vi "UDP test Half 2.vi"() -> ()   [LabVIEW 2013, in "TEC tests.lvlib"]
uses:
  TEC tests.lvlib
  configuration/TEC configuration.lvclass
  execution/TEC runtime.lvclass
  <vilib>/NI/Module Timing Source/usec timing source/usec timing source.lvclass
  configuration/TEC configuration.lvclass/TEC configuration.ctl
  <vilib>/NI/Tag Bus/table/data polymorphs/read one/read Double.vi
  <vilib>/NI/Tag Bus/table/data polymorphs/read one/read Array of U64.vi
  configuration/Write receive on port.vi
  configuration/Write send from port.vi
  configuration/Write send to address.vi
  configuration/Write send to port.vi
  <vilib>/NI/Tag Bus/table/data table.lvlib
  <vilib>/ptbypt/NI_PtbyPt.lvlib
  <vilib>/NI/Configuration Framework/serializable configuration/NISE_CEF_serializable configuration.lvclass
panel:
  out "value":u64[](array[numeric])
  out "error out 2":errorcluster
  out "error out":errorcluster
  in  "send to address":string="dsmith"
  out "duration avg":dbl
  in  "dt":u32=100
  out "duration":dbl
  out "timeout count":u16
  out "final":errorcluster
  out "value rx":dbl
  in  "stop":bool
  out "init err":errorcluster
  in  "ch count":i32=100
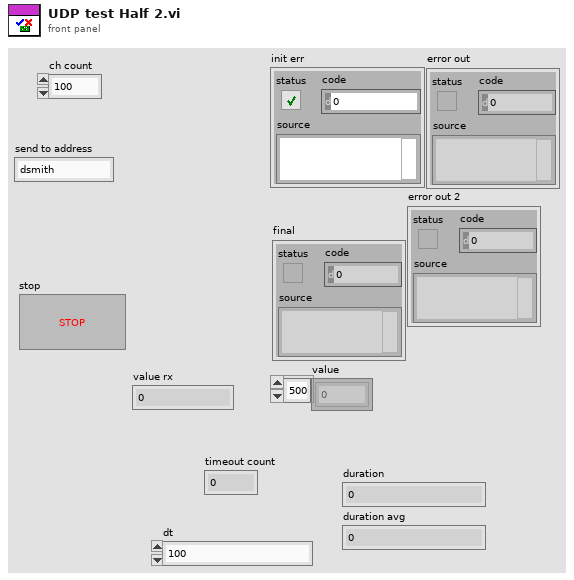
[diagram p1: front panel]
types:
  T1 = typedef "TBM channel.lvclass/data tables.ctl" = cluster{"input data":T2, "processing parameter":T2, "processing result":T2, "output data":T2}
  T2 = typedef "tag bus.lvlib/dictionary table pair.ctl" = cluster{"data dictionary":refnum<class "data dictionary.lvclass">, "data table":T3}
  T3 = typedef "tag bus.lvlib/data table.lvlib/data table.ctl" = cluster{"Double":dbl[], "Single":sgl[], "I64":i64[], "I32":i32[], "I16":i16[], "I8":i8[], "U64":u64[], "U32":u32[], "U16":u16[], "U8":u8[], "Boolean":bool[], "String":string[], "Array of Double":cluster{"DBL Array":dbl[]}[], "Array of Single":cluster{"SGL Array":sgl[]}[], "Array of I64":cluster{"I64 Array":i64[]}[], "Array of I32":cluster{"I32 Array":i32[]}[], "Array of I16":cluster{"I16 Array":i16[]}[], "Array of I8":cluster{"I8 Array":i8[]}[], "Array of U64":cluster{"U64 Array":u64[]}[], "Array of U32":cluster{"U32 Array":u32[]}[], "Array of U16":cluster{"U16 Array":u16[]}[], "Array of U8":cluster{"U8 Array":u8[]}[], "Array of Boolean":cluster{"Boolean Array":bool[]}[], "Array of String":cluster{"String Array":string[]}[]}
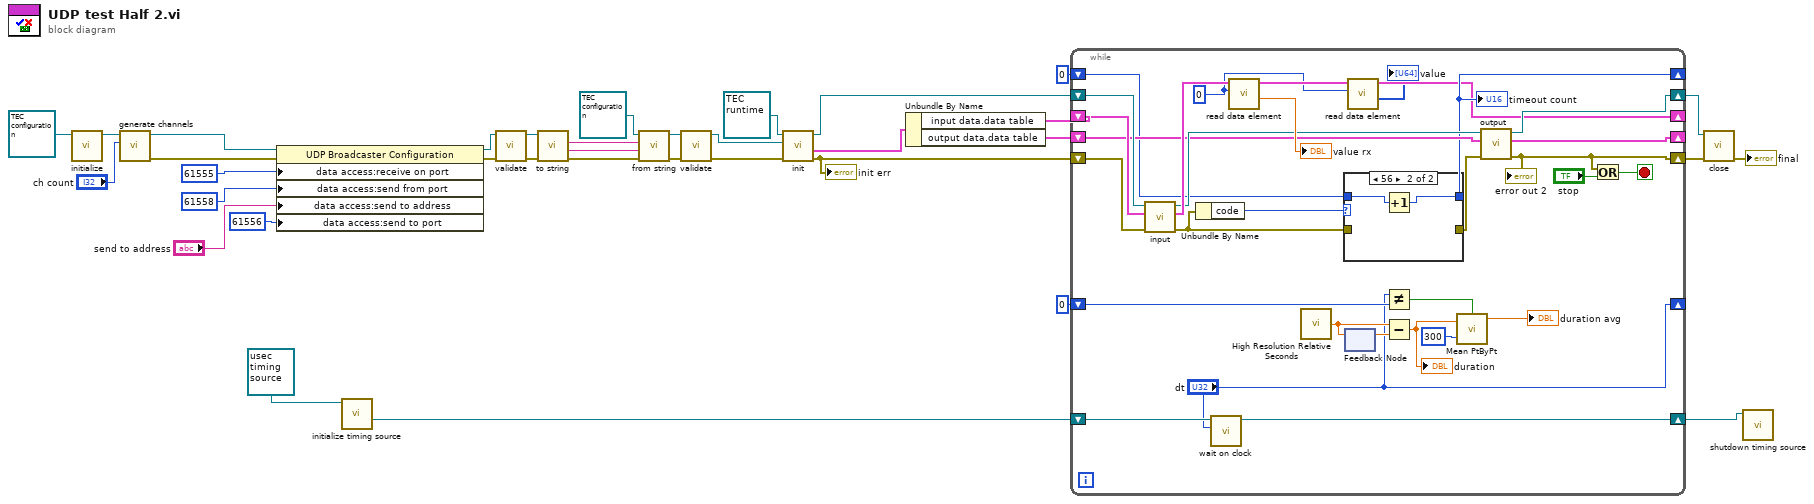
[diagram p0: block diagram]
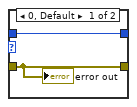
[diagram p2: hidden frame]
diagram:
  n1 = call <vilib>:"initialize.vi"("configuration in"=refnum<class "TEC configuration.lvclass"> refnum ("tag bus configurable plugin module configuration")) -> ("configuration out"=w5:refnum<class "TEC configuration.lvclass">)  [unwired: 8 in, 2 out]
  n2 = call "generate channels.vi"("ch count"="ch count", "TEC configuration in"=w5) -> ("error out"=w7:errorcluster, "TEC configuration out"=w6:refnum<class "TEC configuration.lvclass">)  [unwired: 8 in]
  n3 = property class="UDP Broadcaster Configuration"(reference=w6, error in=w7, "data access:receive on port"=u16 61555 ("send from port"), "data access:send from port"=u16 61558 ("send to port"), "data access:send to address"="send to address", "data access:send to port"=u16 61556 ("receive on port")) -> (reference out=w23:refnum<class "TEC configuration.lvclass">, error out=w24:errorcluster)
  n4 = call-dynamic "initialize timing source.vi"("timing source in"=refnum<class "usec timing source.lvclass"> refnum ("usec timing source.lvclass")) -> ("timing source out"=w2:refnum<class "usec timing source.lvclass">)  [unwired: 9 in, 1 out]
  n5 = call-dynamic "validate.vi"("error in"=w24, "TEC configuration in"=w23) -> ("error out"=w25:errorcluster, "TEC configuration out"=w31:refnum<class "TEC configuration.lvclass">)  [unwired: 8 in]
  n6 = call-dynamic "to string.vi"("error in"=w25, "TEC configuration in"=w31) -> ("error out"=w28:errorcluster, "data"=w27:string, "version"=w26:string)  [unwired: 6 in, 1 out]
  n7 = call-dynamic "from string.vi"("error in"=w28, "data"=w27, "version"=w26, "TEC configuration in"=refnum<class "TEC configuration.lvclass"> refnum) -> ("error out"=w30:errorcluster, "TEC configuration out"=w29:refnum<class "TEC configuration.lvclass">)  [unwired: 6 in]
  n8 = call-dynamic "validate.vi"("error in"=w30, "TEC configuration in"=w29) -> ("error out"=w21:errorcluster, "TEC configuration out"=w20:refnum<class "TEC configuration.lvclass">)  [unwired: 8 in]
  n9 = call-dynamic "init.vi"("error in"=w21, "TBM module configuration in"=w20, "TEC runtime in"=refnum<class "TEC runtime.lvclass"> refnum ("tag bus configurable plugin module")) -> ("error out"=w19:errorcluster, "data allocations"=w17:T1, "TEC runtime out"=w14:refnum<class "TEC runtime.lvclass">)  [unwired: 5 in, 1 out]
  "init err" <- w19
  n10 = Unbundle By Name(w17) -> ("input data.data table"=w16:T3, "output data.data table"=w15:T3)
  n11 = while {
    shift-right: [w41] -> _
    shift-left: w16 -> [w60]
    shift-right: [w56] -> _
    shift-left: w15 -> [w54]
    shift-right: [w57] -> w11
    shift-left: w14 -> [w62]
    shift-right: [w55] -> w13
    shift-left: w19 -> [w61]
    shift-right: [w50] -> _
    shift-left: u16 0 ("Numeric") -> [w49]
    shift-right: ["dt"] -> _
    shift-left: u32 0 ("millisecond multiple") -> [w44]
    shift-right: [w37] -> w1
    shift-left: w2 -> [w38]
    stop <- w65 stop-if-true
    w40 = 0 ("index")
    n12 = call-dynamic "input.vi"("error in"=w61, "data table in"=w60, "TEC runtime in"=w62) -> ("error out"=w52:errorcluster, "data table out"=w59:T3, "TEC runtime out"=w58:refnum<class "TEC runtime.lvclass">)  [unwired: 6 in]
    n13 = Unbundle By Name(w52) -> ("code"=w53:i32)
    n14 = call-dynamic "wait on clock.vi"("dt"="dt", "timing source in"=w38) -> ("timing source out"=w37:refnum<class "usec timing source.lvclass">)  [unwired: 7 in, 2 out]
    n15 = call-poly <vilib>:"read data element.vi"("index"=w40, "data table in"=w59) -> ("value"=→"value rx":dbl, "data table out"=w64:T3)  [unwired: 8 in]
    n16 = call <vilib>:"High Resolution Relative Seconds.vi"() -> ("relative seconds"=w47:dbl)
    n17 = case shown="56" w53 {
      tunnel: w52 -> [w67 _]
      tunnel: [w67 _] -> w51
      tunnel: [w68 w70] -> w50
      tunnel: w49 -> [w68 w69]
      frame 0, Default {
        "error out" <- w67
      }
      frame 56 {
        n18 = Increment(x=w69) -> (x+1=w70:u16)
      }
    }
    "timeout count" <- w50
    n19 = feedback-in #1(w47) -> ()
    n20 = feedback #1() -> (w48:dbl)  [unwired: 1 in]
    n21 = call-poly <vilib>:"read data element.vi"("index"=w40, "data table in"=w64) -> ("value"=→"value":u64[], "data table out"=w41:T3)  [unwired: 8 in]
    n22 = Not Equal?(x="dt", y=w44) -> (x != y?=w43:bool)
    n23 = Subtract(x=w47, y=w48) -> (x-y=w46:dbl)
    "duration" <- w46
    n24 = call <vilib>:"Mean PtByPt.vi"("x"=w46, "sample length"=300, "initialize"=w43) -> ("mean"=→"duration avg":dbl)  [unwired: 1 in, 1 out]
    n25 = call-dynamic "output.vi"("error in"=w51, "data table in"=w54, "TEC runtime in"=w58) -> ("error out"=w55:errorcluster, "data table out"=w56:T3, "TEC runtime out"=w57:refnum<class "TEC runtime.lvclass">)  [unwired: 6 in]
    "error out 2" <- w55
    n26 = Or(x=w55, y="stop") -> (x .or. y?=w65:bool)
  }
  n27 = call-dynamic "close.vi"("error in"=w13, "TEC runtime in"=w11) -> ("error out"=→"final":errorcluster)  [unwired: 9 in]
  n28 = call-dynamic "shutdown timing source.vi"("timing source in"=w1) -> ()  [unwired: 9 in, 2 out]
